vi "CSE - Abort Script Execution.vi"(6 "error in":errorcluster, 7 "action":i32(ring) items=["trigger", "reset", "check", "flip"], 9 "CSE RefNum":T1) -> (0 "error out":errorcluster, 1 "triggered":bool, 3 "dup CSE RefNum":T1)   [LabVIEW 2021]
doc: "This VI aborts execution of the script associated with a specified <b>CSE RefNum</b>. Refer to the VI help for more details.\n\n::: CalcExpress Toolkit :::\nCopyright (c) 2000-2026 Konstantin Shifershteyn. All rights reserved."
uses:
  CSE Instance RefNum.ctl
  cersrc/celveng32.dll
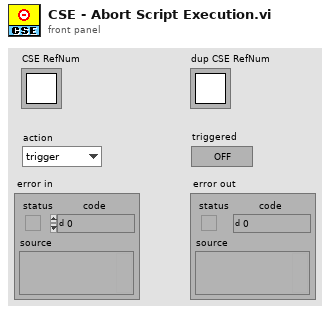
[diagram p1: front panel]
types:
  T1 = typedef "CSE Instance RefNum.ctl" = refnum<k1>
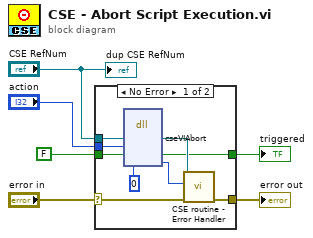
[diagram p0: block diagram]
diagram:
  n1 = case shown="No Error" "error in" {
    selector: "error in" -> [w12 w17]
    tunnel: "CSE RefNum" -> [w14 _]
    tunnel: [w15 w17] -> w6
    tunnel: "action" -> [w9 _]
    tunnel: FALSE -> [w8 w16]
    tunnel: [w7 w16] -> w2
    frame No Error {
      n2 = dll-call lib="C:/LV Projects/CalcExpress 40 LV2021/vi.lib/addons/CalcExpress/cersrc/celveng*.dll" fn="cseVIAbort" ("viCESPAbort")("iRef"=w14, "action"=w9, "state"=w8, "erStat"=0) -> ("iRef"=w13:T1, "state"=w7:bool, "erStat"=w11:i32)  [unwired: 5 in, 2 out]
      n3 = call "CSE routine - Error Handler.vi"("error in"=w12, "exec status"=w11, "CSE RefNum"=w13) -> ("error out"=w15:errorcluster)  [unwired: 4 in, 2 out]
    }
    frame Error {
    }
  }
  "error out" <- w6
  "triggered" <- w2
  "dup CSE RefNum" <- "CSE RefNum"
